vi "XY Sample Stage.vi"(7 "Calling VI Ref":refnum<vi>) -> ()   [LabVIEW 2021]
uses:
  <vilib>/Utility/miscctls.llb/LVPointTypeDef.ctl
  XY Sample Stage Controls/XY Sample Stage History Actions.ctl
  XY Sample Stage Controls/XY Sample Stage XY Settings.ctl
  Hardware Configuration/Hardware Configuration Controls/Device Function.ctl
  Hardware Configuration/Hardware Configuration Controls/Device Type.ctl
  Device Library/Stages/Stages Controls/Stage Actions.ctl
panel:
  in  "Servo On/Off":bool
  in  "Main Tabs":enum32{"XY Control", "Settings"}(tab)
  in  "Up":bool
  in  "Halt":bool
  in  "Down":bool
  in  "Left":bool
  in  "Right":bool
  in  "Home":bool
  in  "X Position (µm)":dbl format="%#_5g"
  in  "Y Position (µm)":dbl format="%#_4g"
  in  "XY Step Size (µm)":dbl format="%#_4g"
  in  "Mark Point":bool
  in  "Clear Points":bool
  in  "Marked Positions":i32(listbox)
  out "Position History":cluster{dbl[], dbl[]}[](graph)
  in  "Scale Factor":dbl
  in  "Active Stage":i32(ring) items=["PI-Stage-Sample XY-COM9", "PI-Stage-Sample Z-E-816", "ASI-Stage-Adj Cavity-COM6", "PI-Stage-Sample Coarse Z-COM3", "PI-Stage-Objective Z-COM10", "PI-Stage-Objective XY-1"]
  in  "Velocity":dbl min=0.0 max=25.0
  in  "Flip X and Y":bool
  in  "Invert X":bool
  in  "Invert Y":bool
  in  "Save XY Config":bool
  in  "Apply Offset":bool
  in  "X Offset":dbl
  in  "Y Offset":dbl
  in  "Quit":bool
  # "Apply Offset to Marked Positions"
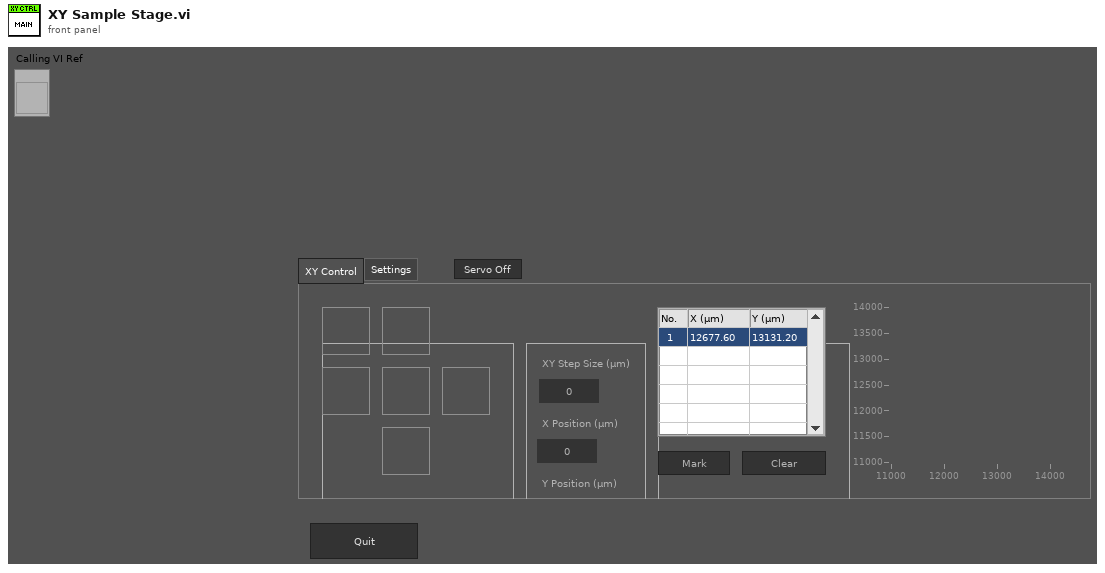
[diagram p1: front panel]
types:
  T1 = typedef "XY Sample Stage XY Settings.ctl" = cluster{"Flip X and Y":bool, "Invert X":bool, "Invert Y":bool}
  T2 = typedef "XY Sample Stage History Actions.ctl" = enum16{"Reset", "Write", "Read", "Set Zero"}
  T3 = enum16{"Always On", "Always Off", "Off While Running"}
  T4 = typedef "LVPointTypeDef.ctl" = cluster{"Horizontal":i16, "Vertical":i16}
  T5 = typedef "LVRectTypeDef.ctl" = cluster{"Left":i16, "Top":i16, "Right":i16, "Bottom":i16}
  T6 = typedef "LVBoundsTypeDef.ctl" = cluster{"Width":u32, "Height":u32}
  T7 = typedef "Stage Actions.ctl" = enum16{"Get Position", "SERVO OFF", "SERVO ON", "SERVO ON/OFF", "MVR", "MOVE", "HALT", "ONTARGET", "ERROR", "REFERENCE", "INIT", "VELOCITY", "STATUS", "EXIT", "HOME", "ZEROPOS", "NANOPOS", "ANALOG", "QUIT"}
  T8 = typedef "Device Type.ctl" = enum16{"AOTF", "Camera", "Deformable Mirror", "Laser", "Flip Mirror", "Shutter", "Stage", "Waveform", "FPGA", "Filter Wheel", "Email"}
  T9 = typedef "Device Function.ctl" = enum16{"Primary", "Secondary", "Overview", "Wide Field Drift Correction", "642 nm Excitation", "560 nm Excitation", "940 nm Excitation", "546 nm Excitation", "488 nm Excitation", "405 nm Excitation", "Objective Drift Correction", "4Pi Focus Lock", "4Pi Objective Lock", "Objective XY", "Objective Z", "Sample XY", "Sample Coarse Z", "Sample Z", "4Pi Lower", "4Pi Upper", "Em Small", "Em Large", "Ex Small", "Ex Large", "Mojo", "Adj Cavity", "Line Scanning", "Alert"}
  T10 = enum8{"Enabled", "Disabled", "Disabled and Grayed Out"}
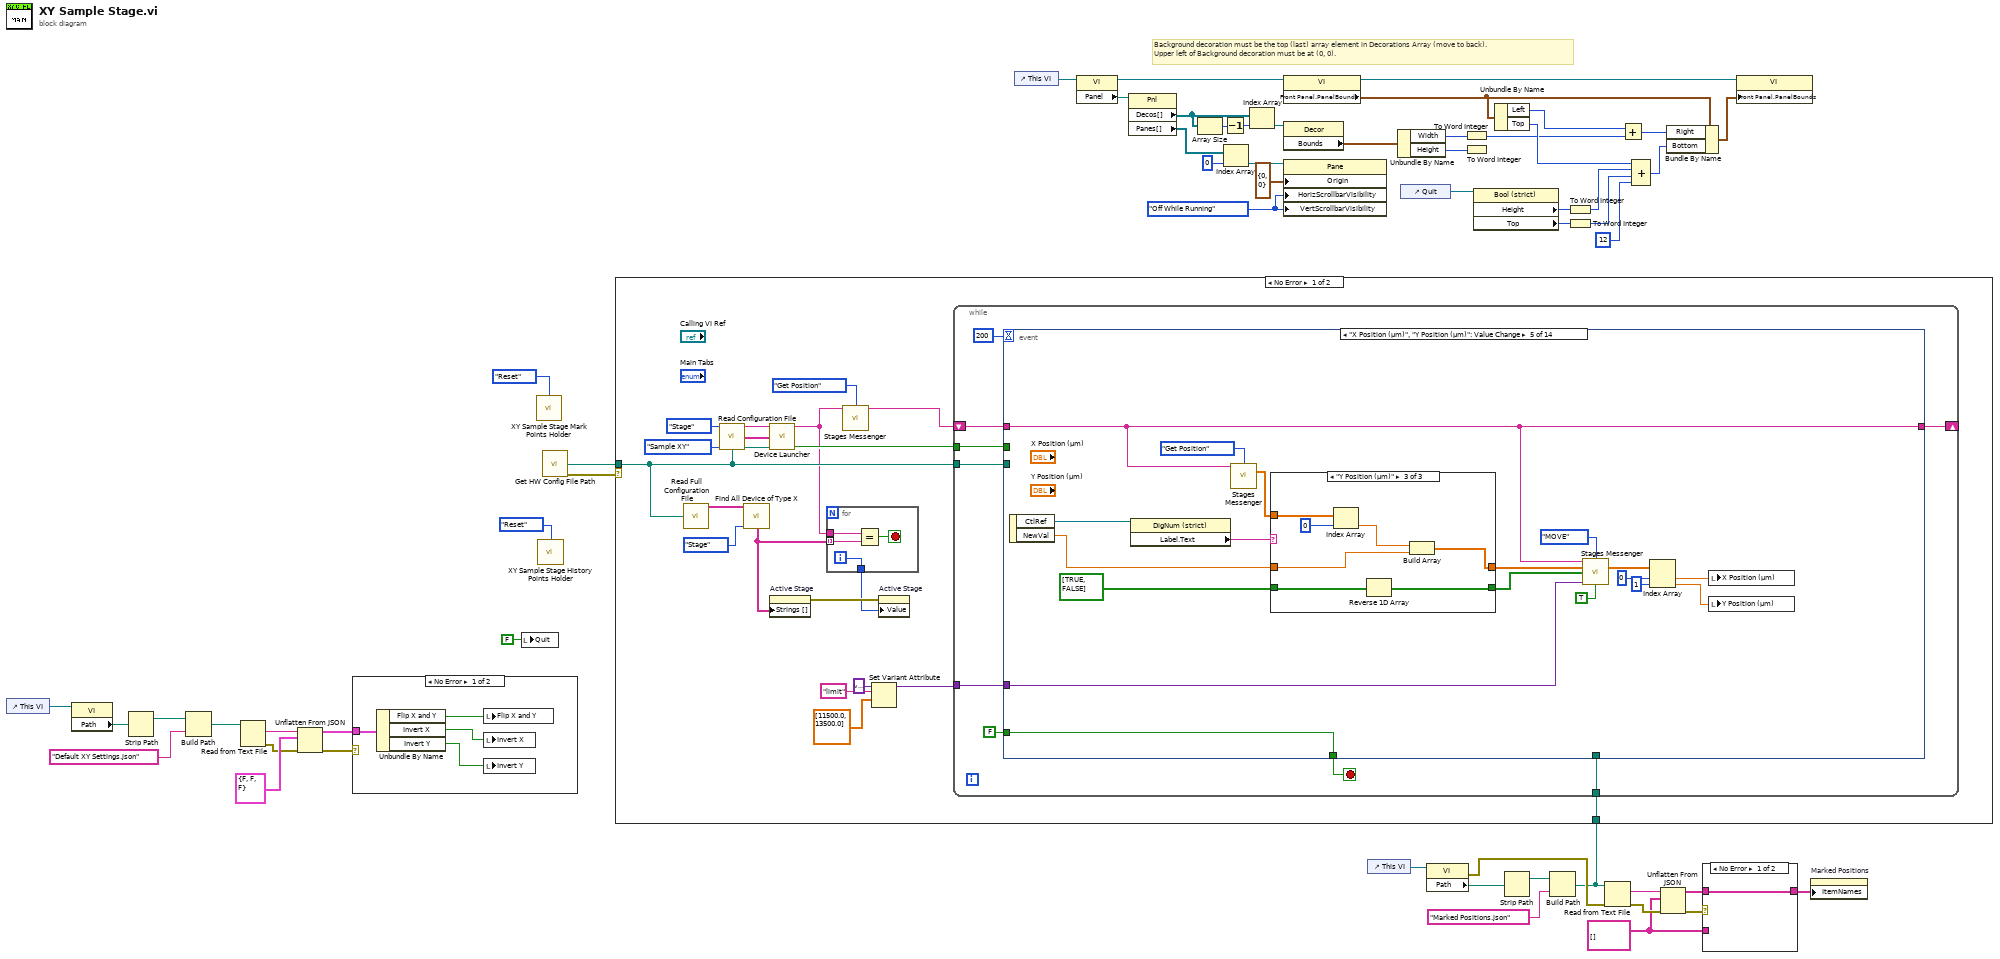
[diagram p0: block diagram]
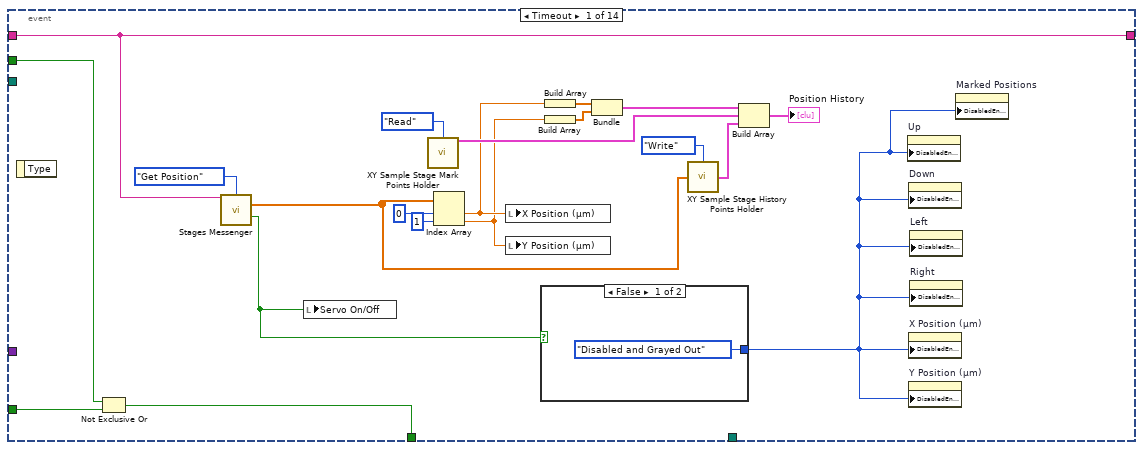
[diagram p4: hidden frame]
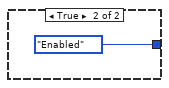
[diagram p5: hidden frame]
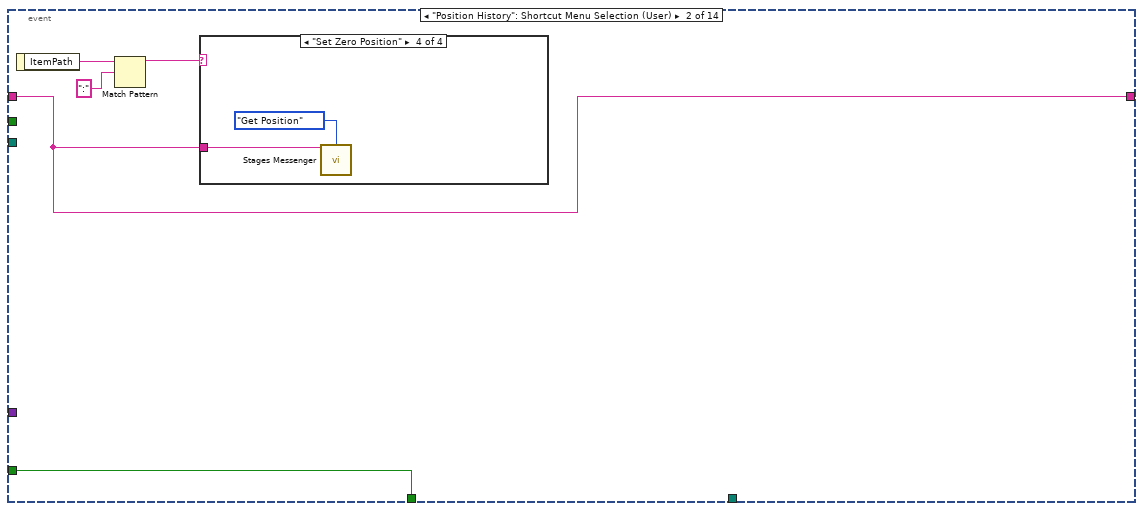
[diagram p6: hidden frame]
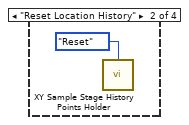
[diagram p8: hidden frame]
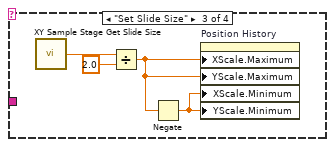
[diagram p9: hidden frame]
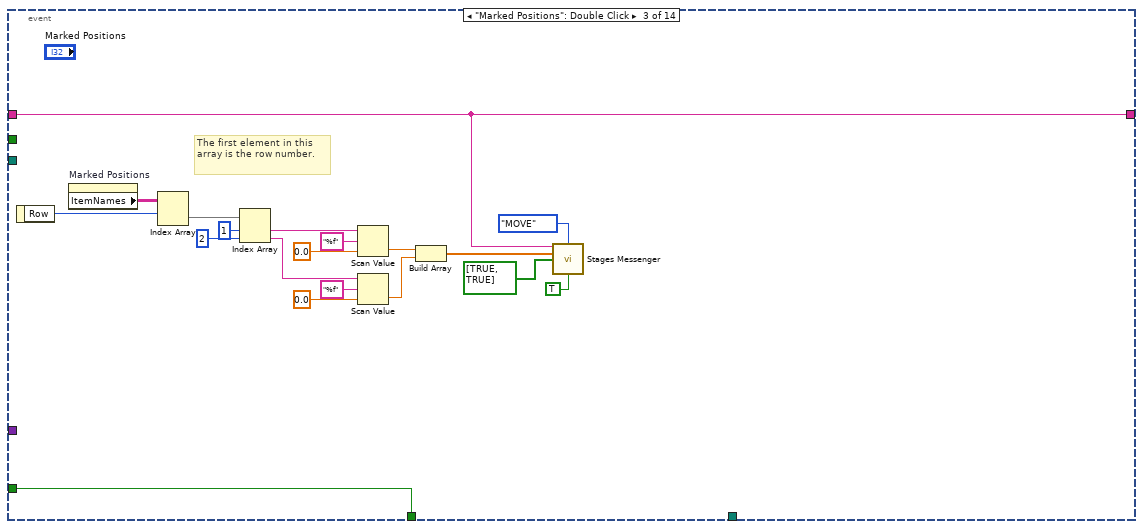
[diagram p10: hidden frame]
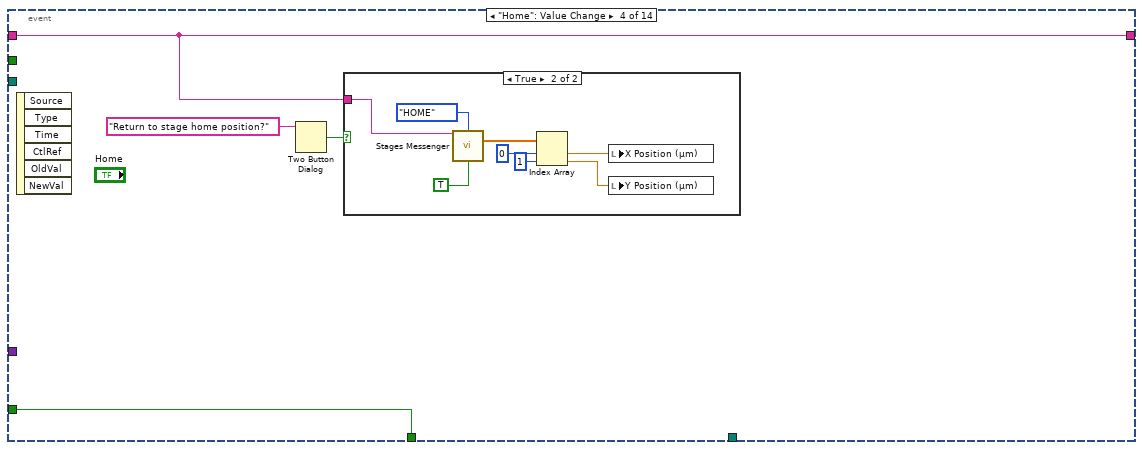
[diagram p11: hidden frame]
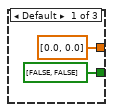
[diagram p13: hidden frame]
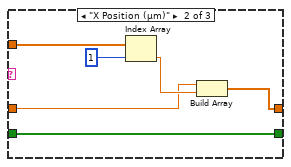
[diagram p14: hidden frame]
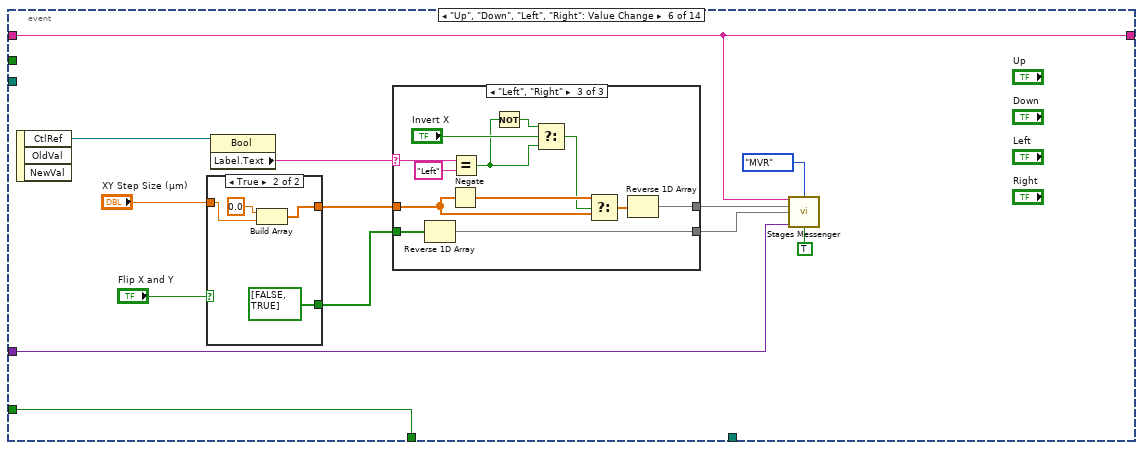
[diagram p15: hidden frame]
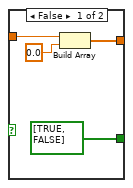
[diagram p16: hidden frame]
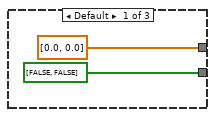
[diagram p17: hidden frame]
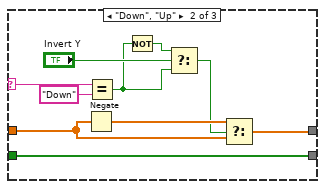
[diagram p18: hidden frame]
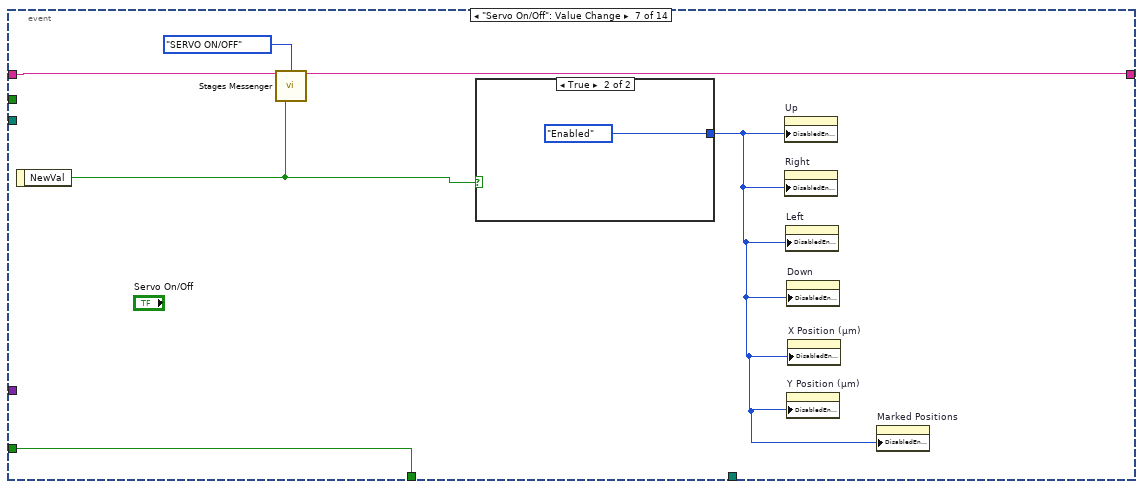
[diagram p19: hidden frame]
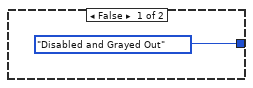
[diagram p20: hidden frame]
diagram:
  w2 = string[][] [] ("Item Names")
  w39 = T3."Off While Running" ("Vertical Scrollbar Visibility")
  # "Background decoration must be the top (last) array element in Decorations Array (move to back).\nUpper left of Background decoration must be at (0, 0)."
  n1 = control-ref of="This VI"() -> (w19:refnum<vi>)
  n2 = property class="VI"(reference=w19) -> ("Path"=w20:path)  [unwired: 1 in, 2 out]
  n3 = Strip Path(path=w20) -> (stripped path=w21:path)  [unwired: 1 out]
  n4 = Build Path(base path=w21, name or relative path="Default XY Settings.json") -> (appended path=w18:path)
  n5 = Read from Text File(file (use dialog)=w18) -> (text=w17:string, error out=w15:errorcluster)  [unwired: 3 in, 2 out]
  n6 = Unflatten From JSON(JSON string=w17, type and defaults=T1 {"Flip X and Y"=FALSE, "Invert X"=FALSE, "Invert Y"=FALSE} ("XY Flip Defaults"), error in (no error)=w15) -> (value=w13:T1, error out=w14:errorcluster)  [unwired: 4 in]
  n7 = case shown="No Error" w14 {
    tunnel: w13 -> [w60 _]
    frame No Error {
      n8 = Unbundle By Name(w60) -> ("Flip X and Y"=w59:bool, "Invert X"=w58:bool, "Invert Y"=w57:bool)
      n9 = local write "Flip X and Y"(w59) -> ()
      n10 = local write "Invert X"(w58) -> ()
      n11 = local write "Invert Y"(w57) -> ()
    }
    frame Error {
    }
  }
  n12 = local write "Quit"(FALSE ("Quit")) -> ()
  n13 = call "XY Sample Stage Mark Points Holder.vi"("Actions"=XY_Sample_Stage_History_Actions."Reset") -> ()  [unwired: 14 in, 1 out]
  n14 = call "XY Sample Stage History Points Holder.vi"("Actions"=XY_Sample_Stage_History_Actions."Reset") -> ()  [unwired: 14 in, 1 out]
  n15 = call "Get HW Config File Path.vi"() -> ("File Path"=w25:path, "Error"=w26:errorcluster)  [unwired: 14 in]
  n16 = control-ref of="This VI"() -> (w31:refnum<vi>)
  n17 = property class="VI"(reference=w31) -> (reference out=w40:refnum<vi>, "Panel"=w32:refnum<vi>)  [unwired: 1 in, 1 out]
  n18 = property class="Pnl"(reference=w32) -> ("Decos[]"=w30:refnum<vi>[], "Panes[]"=w36:refnum<vi>[])  [unwired: 1 in, 2 out]
  n19 = Array Size(array=w30) -> (size(s)=w28:i32)
  n20 = Decrement(x=w28) -> (x-1=w29:i32)
  n21 = Index Array(array=w36, index=0) -> (element=w35:refnum<vi>)
  n22 = Index Array(array=w30, index=w29) -> (element=w38:refnum<vi>)
  n23 = property class="VI"(reference=w40) -> (reference out=w42:refnum<vi>, "Front Panel.PanelBounds"=w43:T5)  [unwired: 1 in, 1 out]
  n24 = property class="Decor"(reference=w38) -> ("Bounds"=w41:T6)  [unwired: 1 in, 2 out]
  n25 = property class="Pane"(reference=w35, "Origin"=T4 {"Horizontal"=0, "Vertical"=0}, "HorizScrollbarVisibility"=w39, "VertScrollbarVisibility"=w39) -> ()  [unwired: 1 in, 2 out]
  n26 = control-ref of="This VI"() -> (w12:refnum<vi>)
  n27 = Unbundle By Name(w41) -> ("Width"=w46:u32, "Height"=w49:u32)
  n28 = control-ref of="Quit"() -> (w33:refnum<vi>)
  n29 = property class="VI"(reference=w12) -> (error out=w7:errorcluster, "Path"=w11:path)  [unwired: 1 in, 1 out]
  n30 = To Word Integer(number=w46) -> (16bit integer=w48:i16)
  n31 = To Word Integer(number=w49) -> ()  [unwired: 1 out]
  n32 = property class="Bool (strict)"(reference=w33) -> ("Height"=w51:u32, "Top"=w52:i32)  [unwired: 1 in, 2 out]
  n33 = Unbundle By Name(w43) -> ("Left"=w45:i16, "Top"=w56:i16)
  n34 = Strip Path(path=w11) -> (stripped path=w10:path)  [unwired: 1 out]
  n35 = Build Path(base path=w10, name or relative path="Marked Positions.json") -> (appended path=w1:path)
  n36 = case shown="No Error" w26 {
    tunnel: w25 -> [w69 _]
    tunnel: w1 -> [w65 _]
    frame No Error {
      n37 = call "Read Full Configuration File.vi"("Config File Path"=w69) -> ("Unique Notifier Names"=w74:string[])  [unwired: 11 in, 3 out]
      n38 = call "Read Configuration File.vi"("Device Type"=Device_Type."Stage", "Device Function"=Device_Function."Sample XY", "Config File Path"=w69) -> ("Unique Notifier Name"=w80:string, "Device Ports/IDs/Channels"=w78:string[], "Device Engine Path"=w79:path)  [unwired: 9 in, 1 out]
      n39 = call "Find All Device of Type X.vi"("Unique Notifier Names"=w74, "Device Type"=Device_Type."Stage") -> ("All Devices"=w72:string[])  [unwired: 12 in, 1 out]
      n40 = call "Device Launcher.vi"("Notifier Name"=w80, "Device Ports/IDs/Channels"=w78, "Device Engine Path"=w79) -> ("Notifier Name"=w67:string, "Running?"=w75:bool)  [unwired: 11 in]
      n41 = property on="Active Stage" class="Ring (strict)"("Strings []"=w72) -> (error out=w71:errorcluster)  [unwired: 2 in, 1 out]
      n42 = for {
        tunnel: w72 -> [w83] mode=indexing
        tunnel: w67 -> [w84]
        tunnel: [w81] -> w70
        i -> [w81]
        stop <- w82 stop-if-true
        n43 = Equal?(x=w84, y=w83) -> (x = y?=w82:bool)
      }
      n44 = call "Stages Messenger.vi"("Stage Notifier Name"=w67, "Actions"=Stage_Actions."Get Position") -> ("Stage Notifier Name (Dup)"=w66:string)  [unwired: 9 in, 4 out]
      n45 = Set Variant Attribute(Variant=variant ("variant"), name="limit", value=dbl[] [11500.0, 13500.0] ("Array")) -> (Variant out=w61:variant)  [unwired: 1 in, 2 out]
      n46 = property on="Active Stage" class="Ring (strict)"(error in=w71, "Value"=w70) -> ()  [unwired: 1 in, 2 out]
      n47 = while {
        tunnel: w75 -> [w90]
        shift-right: [w88] -> _
        shift-left: w66 -> [w91]
        tunnel: w69 -> [w87]
        tunnel: w65 -> [w86]
        tunnel: w61 -> [w85]
        stop <- w93 stop-if-true
        n48 = event shown="[4] \"X Position (µm)\", \"Y Position (µm)\": Value Change" {
          selector: _ -> [_ _ _ _ _ _ _ _ _ _ _ _ _ _]
          dyn-events: _ -> [_ _ _ _ _ _ _ _ _ _ _ _ _ _]
          timeout: 200 -> [_ _ _ _ _ _ _ _ _ _ _ _ _ _]
          tunnel: [w99 w118 w146 w150 w176 w204 w239 w247 w255 w282 w295 w307 w322 TRUE ("NewVal")] -> w93
          tunnel: FALSE ("NewVal") -> [w100 w118 w146 w150 w176 w204 w239 w247 w255 w282 w295 w307 w322 _]
          tunnel: w91 -> [w98 w116 w129 w147 w161 w193 w242 w246 w252 w281 w283 _ w317 w349]
          tunnel: w90 -> [w101 _ _ _ _ _ _ _ _ _ _ _ _ _]
          tunnel: [w98 w116 w129 w147 w161 w193 w238 w245 w252 w278 w283 w296 w317 w349] -> w88
          tunnel: w87 -> [_ _ _ _ _ _ _ _ _ _ _ w305 _ _]
          tunnel: w86 -> [_ _ _ _ _ _ _ _ w249 _ _ _ _ _]
          tunnel: w85 -> [_ _ _ _ w163 w192 _ _ _ _ _ _ _ _]
          event Timeout {
            n49 = event-data() -> ()  [unwired: 1 in, 1 out]
            n50 = Not Exclusive Or(1:w100, 2:w101) -> (0:w99:bool)
            n51 = call "Stages Messenger.vi"("Stage Notifier Name"=w98, "Actions"=Stage_Actions."Get Position") -> ("Positions"=w105:dbl[], "Servo Status"=w95:bool)  [unwired: 9 in, 3 out]
            n52 = local write "Servo On/Off"(w95) -> ()
            n53 = call "XY Sample Stage Mark Points Holder.vi"("Actions"=XY_Sample_Stage_History_Actions."Read") -> ("Marked Points"=w102:cluster{dbl[], dbl[]})  [unwired: 14 in]
            n54 = Index Array(array=w105, index #1=0 ("index"), index #2=1 ("index")) -> (element #1=w97:dbl, element #2=w96:dbl)
            n55 = local write "X Position (µm)"(w97) -> ()
            n56 = local write "Y Position (µm)"(w96) -> ()
            n57 = case shown="False" w95 {
              tunnel: [T10."Disabled and Grayed Out" ("Disabled") T10."Enabled" ("Disabled")] -> w94
              frame False {
              }
              frame True {
              }
            }
            n58 = Build Array(w97) -> (w110:dbl[])
            n59 = Build Array(w96) -> (w109:dbl[])
            n60 = Bundle(w110, w109) -> (w103:cluster{dbl[], dbl[]})  [unwired: 1 in]
            n61 = call "XY Sample Stage History Points Holder.vi"("Actions"=XY_Sample_Stage_History_Actions."Write", "(x, y) Points"=w105) -> ("History Points"=w108:cluster{dbl[], dbl[]})  [unwired: 13 in]
            n62 = Build Array(w103, w102, w108) -> (→"Position History":cluster{dbl[], dbl[]}[])
            n63 = property on="Up" class="Bool"("DisabledEnum"=w94) -> ()  [unwired: 2 in, 2 out]
            n64 = property on="Down" class="Bool"("DisabledEnum"=w94) -> ()  [unwired: 2 in, 2 out]
            n65 = property on="X Position (µm)" class="DigNum (strict)"("DisabledEnum"=w94) -> ()  [unwired: 2 in, 2 out]
            n66 = property on="Y Position (µm)" class="DigNum (strict)"("DisabledEnum"=w94) -> ()  [unwired: 2 in, 2 out]
            n67 = property on="Left" class="Bool"("DisabledEnum"=w94) -> ()  [unwired: 2 in, 2 out]
            n68 = property on="Right" class="Bool"("DisabledEnum"=w94) -> ()  [unwired: 2 in, 2 out]
            n69 = property on="Marked Positions" class="MCListbox (strict)"("DisabledEnum"=w94) -> ()  [unwired: 2 in, 2 out]
          }
          event "Position History": Shortcut Menu Selection (User) {
            n70 = event-data() -> ("ItemPath"=w119:string)  [unwired: 1 in]
            n71 = Match Pattern(string=w119, regular expression=":") -> (before substring=w117:string)  [unwired: 1 in, 3 out]
            n72 = case shown="\"Set Zero Position\"" w117 {
              tunnel: w116 -> [_ _ _ w126]
              frame Default {
              }
              frame "Reset Location History" {
                n73 = call "XY Sample Stage History Points Holder.vi"("Actions"=XY_Sample_Stage_History_Actions."Reset") -> ()  [unwired: 14 in, 1 out]
              }
              frame "Set Slide Size" {
                n74 = call "XY Sample Stage Get Slide Size.vi"() -> ("Slide Size Out mm)"=w125:dbl)  [unwired: 15 in]
                n75 = Divide(x=w125, y=2.0) -> (x/y=w123:dbl)
                n76 = Negate(x=w123) -> (-x=w122:dbl)
                n77 = property on="Position History" class="XYGraph (strict)"("XScale.Maximum"=w123, "YScale.Maximum"=w123, "XScale.Minimum"=w122, "YScale.Minimum"=w122) -> ()  [unwired: 2 in, 2 out]
              }
              frame "Set Zero Position" {
                n78 = call "Stages Messenger.vi"("Stage Notifier Name"=w126, "Actions"=Stage_Actions."Get Position") -> ()  [unwired: 9 in, 5 out]
              }
            }
          }
          event "Marked Positions": Double Click {
            # "The first element in this array is the row number."
            n79 = event-data() -> ("Row"=w144:i32)  [unwired: 1 in]
            n80 = property on="Marked Positions" class="MCListbox (strict)"() -> ("ItemNames"=w145:string[][])  [unwired: 2 in, 2 out]
            n81 = Index Array(array=w145, index (row)=w144) -> (element=w138:string[])  [unwired: 1 in]
            n82 = Index Array(array=w138, index #1=1 ("index"), index #2=2 ("index")) -> (element #1=w133:string, element #2=w128:string)
            n83 = Scan Value(string=w133, format string="%f", default (0 dbl)=0.0) -> (value=w132:dbl)  [unwired: 1 out]
            n84 = Scan Value(string=w128, format string="%f", default (0 dbl)=0.0) -> (value=w131:dbl)  [unwired: 1 out]
            n85 = Build Array(w132, w131) -> (w130:dbl[])
            n86 = call "Stages Messenger.vi"("Stage Notifier Name"=w129, "Actions"=Stage_Actions."MOVE", "Setpoint"=w130, "Axis"=bool[] [TRUE, TRUE], "Exit While Busy?"=TRUE ("Wait for On Target? (F)")) -> ()  [unwired: 6 in, 5 out]
          }
          event "Home": Value Change {
            n87 = event-data() -> ()  [unwired: 1 in, 6 out]
            n88 = Two Button Dialog(message="Return to stage home position?") -> (T button?=w148:bool)  [unwired: 2 in]
            n89 = case shown="True" w148 {
              tunnel: w147 -> [_ w157]
              frame False {
              }
              frame True {
                n90 = call "Stages Messenger.vi"("Stage Notifier Name"=w157, "Actions"=Stage_Actions."HOME", "Exit While Busy?"=TRUE) -> ("Positions"=w152:dbl[])  [unwired: 8 in, 4 out]
                n91 = Index Array(array=w152, index #1=0 ("index"), index #2=1 ("index")) -> (element #1=w154:dbl, element #2=w153:dbl)
                n92 = local write "X Position (µm)"(w154) -> ()
                n93 = local write "Y Position (µm)"(w153) -> ()
              }
            }
          }
          event "X Position (µm)", "Y Position (µm)": Value Change {
            n94 = event-data() -> ("CtlRef"=w175:refnum<vi>, "NewVal"=w159:dbl)  [unwired: 1 in]
            n95 = property class="DigNum (strict)"(reference=w175) -> ("Label.Text"=w174:string)  [unwired: 1 in, 2 out]
            n96 = call "Stages Messenger.vi"("Stage Notifier Name"=w161, "Actions"=Stage_Actions."Get Position") -> ("Positions"=w160:dbl[])  [unwired: 9 in, 4 out]
            n97 = case shown="\"Y Position (µm)\"" w174 {
              tunnel: w159 -> [_ w180 w186]
              tunnel: bool[] [TRUE, FALSE] -> [_ w184 w191]
              tunnel: [dbl[] [0.0, 0.0] w179 w185] -> w171
              tunnel: [bool[] [FALSE, FALSE] w184 w190] -> w170
              tunnel: w160 -> [_ w182 w188]
              frame Default {
              }
              frame "X Position (µm)" {
                n98 = Index Array(array=w182, index=1) -> (element=w181:dbl)
                n99 = Build Array(w180, w181) -> (w179:dbl[])
              }
              frame "Y Position (µm)" {
                n100 = Index Array(array=w188, index=0) -> (element=w187:dbl)
                n101 = Reverse 1D Array(array=w191) -> (reversed array=w190:bool[])
                n102 = Build Array(w187, w186) -> (w185:dbl[])
              }
            }
            n103 = call "Stages Messenger.vi"("Stage Notifier Name"=w161, "Actions"=Stage_Actions."MOVE", "Setpoint"=w171, "Axis"=w170, "Misc"=w163, "Exit While Busy?"=TRUE ("Wait for On Target? (F)")) -> ("Positions"=w164:dbl[])  [unwired: 5 in, 4 out]
            n104 = Index Array(array=w164, index #1=0 ("index"), index #2=1 ("index")) -> (element #1=w166:dbl, element #2=w165:dbl)
            n105 = local write "X Position (µm)"(w166) -> ()
            n106 = local write "Y Position (µm)"(w165) -> ()
          }
          event "Up", "Down", "Left", "Right": Value Change {
            n107 = event-data() -> ("CtlRef"=w203:refnum<vi>)  [unwired: 1 in, 2 out]
            n108 = case shown="True" "Flip X and Y" {
              tunnel: [bool[] [TRUE, FALSE] bool[] [FALSE, TRUE]] -> w197
              tunnel: [w206 w211] -> w195
              tunnel: "XY Step Size (µm)" -> [w205 w210]
              frame False {
                n109 = Build Array(w205, 0.0 ("element")) -> (w206:dbl[])
              }
              frame True {
                n110 = Build Array(0.0 ("element"), w210) -> (w211:dbl[])
              }
            }
            n111 = property class="Bool"(reference=w203) -> ("Label.Text"=w202:string)  [unwired: 1 in, 2 out]
            n112 = case shown="\"Left\", \"Right\"" w202 {
              selector: w202 -> [_ w224 w234]
              tunnel: w195 -> [_ w221 w233]
              tunnel: w197 -> [_ w219 w231]
              tunnel: [dbl[] [0.0, 0.0] w220 w230] -> w199
              tunnel: [bool[] [FALSE, FALSE] w219 w229] -> w198
              frame Default {
              }
              frame "Down", "Up" {
                n113 = Negate(x=w221) -> (-x=w222:dbl[])
                n114 = Equal?(x=w224, y="Down") -> (x = y?=w217:bool)
                n115 = Not(x=w217) -> (.not. x?=w216:bool)
                n116 = Select(t=w216, s="Invert Y", f=w217) -> (s? t:f=w215:bool)
                n117 = Select(t=w222, s=w215, f=w221) -> (s? t:f=w220:dbl[])
              }
              frame "Left", "Right" {
                n118 = Reverse 1D Array(array=w231) -> (reversed array=w229:bool[])
                n119 = Negate(x=w233) -> (-x=w235:dbl[])
                n120 = Equal?(x=w234, y="Left") -> (x = y?=w226:bool)
                n121 = Not(x=w226) -> (.not. x?=w228:bool)
                n122 = Select(t=w228, s="Invert X", f=w226) -> (s? t:f=w225:bool)
                n123 = Select(t=w235, s=w225, f=w233) -> (s? t:f=w232:dbl[])
                n124 = Reverse 1D Array(array=w232) -> (reversed array=w230:dbl[])
              }
            }
            n125 = call "Stages Messenger.vi"("Stage Notifier Name"=w193, "Actions"=Stage_Actions."MVR", "Setpoint"=w199, "Axis"=w198, "Misc"=w192, "Exit While Busy?"=TRUE ("Wait for On Target? (F)")) -> ()  [unwired: 5 in, 5 out]
          }
          event "Servo On/Off": Value Change {
            n126 = event-data() -> ("NewVal"=w240:bool)  [unwired: 1 in]
            n127 = call "Stages Messenger.vi"("Stage Notifier Name"=w242, "Actions"=Stage_Actions."SERVO ON/OFF", "Servo On?"=w240) -> ("Stage Notifier Name (Dup)"=w238:string)  [unwired: 8 in, 4 out]
            n128 = case shown="True" w240 {
              tunnel: [T10."Disabled and Grayed Out" ("Disabled") T10."Enabled" ("Disabled")] -> w237
              frame False {
              }
              frame True {
              }
            }
            n129 = property on="Up" class="Bool"("DisabledEnum"=w237) -> ()  [unwired: 2 in, 2 out]
            n130 = property on="Right" class="Bool"("DisabledEnum"=w237) -> ()  [unwired: 2 in, 2 out]
            n131 = property on="Left" class="Bool"("DisabledEnum"=w237) -> ()  [unwired: 2 in, 2 out]
            n132 = property on="Down" class="Bool"("DisabledEnum"=w237) -> ()  [unwired: 2 in, 2 out]
            n133 = property on="Y Position (µm)" class="DigNum (strict)"("DisabledEnum"=w237) -> ()  [unwired: 2 in, 2 out]
            n134 = property on="X Position (µm)" class="DigNum (strict)"("DisabledEnum"=w237) -> ()  [unwired: 2 in, 2 out]
            n135 = property on="Marked Positions" class="MCListbox (strict)"("DisabledEnum"=w237) -> ()  [unwired: 2 in, 2 out]
          }
          event "Halt": Value Change {
            n136 = event-data() -> ()  [unwired: 1 in, 6 out]
            n137 = call "Stages Messenger.vi"("Stage Notifier Name"=w246, "Actions"=Stage_Actions."HALT") -> ("Stage Notifier Name (Dup)"=w245:string)  [unwired: 9 in, 4 out]
          }
          event "Mark Point", "Clear Points": Value Change {
            n138 = event-data() -> ("CtlRef"=w254:refnum<vi>)  [unwired: 1 in]
            n139 = property class="Bool"(reference=w254) -> ("Label.Text"=w253:string)  [unwired: 1 in, 2 out]
            n140 = case shown="\"Clear Points\", Default" w253 {
              tunnel: [string[][] [] w258] -> w250
              tunnel: w252 -> [_ w259]
              frame "Clear Points", Default {
                n141 = call "XY Sample Stage Mark Points Holder.vi"("Actions"=XY_Sample_Stage_History_Actions."Reset") -> ()  [unwired: 14 in, 1 out]
              }
              frame "Mark Point" {
                w272 = "%.2f" ("format string")
                n142 = property on="Marked Positions" class="MCListbox (strict)"() -> ("ItemNames"=w263:string[][])  [unwired: 2 in, 2 out]
                n143 = call "Stages Messenger.vi"("Stage Notifier Name"=w259, "Actions"=Stage_Actions."Get Position") -> ("Positions"=w261:dbl[])  [unwired: 9 in, 4 out]
                n144 = Array Size(array=w263) -> (size(s)=w269:i32[])
                n145 = Index Array(array=w261, index #1=0 ("index"), index #2=1 ("index")) -> (element #1=w274:dbl, element #2=w273:dbl)
                n146 = Index Array(array=w269, index=0) -> (element=w267:i32)
                n147 = call "XY Sample Stage Mark Points Holder.vi"("Actions"=XY_Sample_Stage_History_Actions."Write", "(X, Y) Points"=w261) -> ()  [unwired: 13 in, 1 out]
                n148 = Increment(x=w267) -> (x+1=w271:i32)
                n149 = Number To Decimal String(number=w271, width (-)=i16 3) -> (decimal integer string=w266:string)
                n150 = Format Value(format string=w272, value (0)=w274) -> (output string=w264:string)  [unwired: 1 in]
                n151 = Format Value(format string=w272, value (0)=w273) -> (output string=w265:string)  [unwired: 1 in]
                n152 = Build Array(w266, w264, w265) -> (w262:string[])
                n153 = Build Array (concatenate)(w263, w262) -> (w258:string[][])
              }
            }
            n154 = Flatten To JSON(anything=w250) -> (JSON string=w251:string)  [unwired: 2 in, 1 out]
            n155 = property on="Marked Positions" class="MCListbox (strict)"("ItemNames"=w250) -> ()  [unwired: 2 in, 2 out]
            n156 = Write to Text File(file (use dialog)=w249, text=w251) -> ()  [unwired: 2 in, 3 out]
          }
          event "Velocity": Value Change {
            n157 = event-data() -> ("NewVal"=w279:dbl)  [unwired: 1 in]
            n158 = call "Stages Messenger.vi"("Stage Notifier Name"=w281, "Actions"=Stage_Actions."VELOCITY", "Velocity"=w279) -> ("Stage Notifier Name (Dup)"=w278:string)  [unwired: 8 in, 4 out]
          }
          event "Save XY Config": Value Change {
            n159 = event-data() -> ()  [unwired: 1 in, 1 out]
            n160 = control-ref of="This VI"() -> (w294:refnum<vi>)
            n161 = local read "Flip X and Y"() -> (w289:bool)
            n162 = local read "Invert X"() -> (w288:bool)
            n163 = local read "Invert Y"() -> (w287:bool)
            n164 = property class="VI"(reference=w294) -> ("Path"=w293:path)  [unwired: 1 in, 2 out]
            n165 = Bundle By Name(cluster=T1 {"Flip X and Y"=FALSE, "Invert X"=TRUE, "Invert Y"=TRUE} ("XY Flip Defaults"), "Flip X and Y"=w289, "Invert X"=w288, "Invert Y"=w287) -> (w286:T1)
            n166 = Strip Path(path=w293) -> (stripped path=w292:path)  [unwired: 1 out]
            n167 = Build Path(base path=w292, name or relative path="Default XY Settings.json") -> (appended path=w285:path)
            n168 = Flatten To JSON(anything=w286) -> (JSON string=w284:string)  [unwired: 2 in, 1 out]
            n169 = Write to Text File(file (use dialog)=w285, text=w284) -> ()  [unwired: 2 in, 3 out]
          }
          event "Active Stage": Value Change {
            n170 = event-data() -> ("CtlRef"=w306:refnum<vi>)  [unwired: 1 in]
            n171 = property class="Ring (strict)"(reference=w306) -> ("RingText.Text"=w304:string)  [unwired: 1 in, 2 out]
            n172 = call "Read Full Configuration File.vi"("Config File Path"=w305) -> ("Unique Notifier Names"=w303:string[], "Device Port/ID/Channel Info"=w302:string[][], "Device Engine Paths"=w301:path[])  [unwired: 11 in, 1 out]
            n173 = for {
              tunnel: w304 -> [w310]
              tunnel: w303 -> [w311] mode=indexing
              tunnel: [w308] -> w300
              i -> [w308]
              stop <- w309 stop-if-true
              n174 = Equal?(x=w311, y=w310) -> (x = y?=w309:bool)
            }
            n175 = Index Array(array=w303, index=w300) -> (element=w299:string)
            n176 = Index Array(array=w302, index (row)=w300) -> (element=w298:string[])  [unwired: 1 in]
            n177 = Index Array(array=w301, index=w300) -> (element=w297:path)
            n178 = call "Device Launcher.vi"("Notifier Name"=w299, "Device Ports/IDs/Channels"=w298, "Device Engine Path"=w297) -> ("Notifier Name"=w296:string)  [unwired: 11 in, 1 out]
          }
          event "Apply Offset": Value Change {
            n179 = event-data() -> ()  [unwired: 1 in, 1 out]
            n180 = property on="Marked Positions" class="MCListbox (strict)"() -> ("ItemNames"=w321:string[][])  [unwired: 2 in, 2 out]
            n181 = Array Size(array=w321) -> (size(s)=w320:i32[])
            n182 = Index Array(array=w320, index=0) -> (element=w318:i32)
            n183 = for {
              N: w318 -> [_]
              tunnel: w321 -> [w348]
              tunnel: [w333] -> w316 mode=indexing
              tunnel: [w329] -> w315 mode=indexing
              tunnel: [w328] -> w314 mode=indexing
              i -> [w334]
              w332 = "%.2f" ("format string")
              n184 = Index Array(array=w348, index (row)=w334) -> (element=w345:string[])  [unwired: 1 in]
              n185 = Increment(x=w334) -> (x+1=w335:i32)
              n186 = Index Array(array=w345, index #1=1 ("index"), index #2=2 ("index")) -> (element #1=w340:string, element #2=w339:string)
              n187 = Number To Decimal String(number=w335, width (-)=i16 3) -> (decimal integer string=w333:string)
              n188 = Scan Value(string=w340, format string="%f", default (0 dbl)=0.0) -> (value=w327:dbl)  [unwired: 1 out]
              n189 = Scan Value(string=w339, format string="%f", default (0 dbl)=0.0) -> (value=w326:dbl)  [unwired: 1 out]
              n190 = Divide(x=w327, y="Scale Factor") -> (x/y=w325:dbl)
              n191 = Divide(x=w326, y="Scale Factor") -> (x/y=w324:dbl)
              n192 = Add(x="X Offset", y=w325) -> (x+y=w331:dbl)
              n193 = Add(x=w324, y="Y Offset") -> (x+y=w330:dbl)
              n194 = Format Value(format string=w332, value (0)=w331) -> (output string=w329:string)  [unwired: 1 in]
              n195 = Format Value(format string=w332, value (0)=w330) -> (output string=w328:string)  [unwired: 1 in]
            }
            n196 = Build Array(w316, w315, w314) -> (w313:string[][])
            n197 = Transpose 2D Array(2D array=w313) -> (transposed array=w312:string[][])
            n198 = property on="Marked Positions" class="MCListbox (strict)"("ItemNames"=w312) -> ()  [unwired: 2 in, 2 out]
          }
          event "Quit": Value Change {
            n199 = event-data() -> ()  [unwired: 1 in, 6 out]
          }
        }
      }
    }
    frame Error {
      n200 = control-ref of="This VI"() -> (w356:refnum<vi>)
      n201 = property class="VI"(reference=w356) -> ("Name"=w354:string)  [unwired: 1 in, 2 out]
      n202 = Concatenate Strings("Error in ", w354, "\r", "No Config File") -> (w351:string)
      n203 = One Button Dialog(message=w351) -> ()  [unwired: 1 in, 1 out]
    }
  }
  n204 = To Word Integer(number=w51) -> (16bit integer=w54:i16)
  n205 = To Word Integer(number=w52) -> (16bit integer=w55:i16)
  n206 = Read from Text File(file (use dialog)=w1, error in=w7) -> (text=w8:string, error out=w6:errorcluster)  [unwired: 2 in, 2 out]
  n207 = Add(x=w45, y=w48) -> (x+y=w47:i16)
  n208 = Compound Arithmetic op=ADD(w56, w54, w55, i16 12 ("y")) -> (w50:i16)
  n209 = Unflatten From JSON(JSON string=w8, type and defaults=w2, error in (no error)=w6) -> (value=w4:string[][], error out=w5:errorcluster)  [unwired: 4 in]
  n210 = Bundle By Name(cluster=w43, "Right"=w47, "Bottom"=w50) -> (w44:T5)
  n211 = case shown="No Error" w5 {
    tunnel: w4 -> [w357 _]
    tunnel: [w357 w358] -> w3
    tunnel: w2 -> [_ w358]
    frame No Error {
    }
    frame Error {
    }
  }
  n212 = property class="VI"(reference=w42, "Front Panel.PanelBounds"=w44) -> ()  [unwired: 1 in, 2 out]
  n213 = property on="Marked Positions" class="MCListbox (strict)"("ItemNames"=w3) -> ()  [unwired: 2 in, 2 out]
